vi "Save to File.vi"(8 "error in":errorcluster, 10 "Folder":path, 11 "ILabVIEWFile in":refnum<class "Type Definition.lvclass">) -> (0 "error out":errorcluster, 2 "File Path":path, 3 "ILabVIEWFile out":refnum<class "Type Definition.lvclass">)   [LabVIEW 2026, in "Type Definition.lvclass"]
doc: "Save object to file at the provided path."
uses:
  Type Definition.lvclass
  C:/Users/juanj/Documents/hasbun_wood_engineering/github/py2vi/labview/Classes/LabVIEW File/LabVIEW File.lvclass
  LabVIEW File/LabVIEW File.lvclass/LabVIEW File.ctl
  LabVIEW File/Read VI Reference.vi
  Type Definition.lvclass/Type Definition.ctl
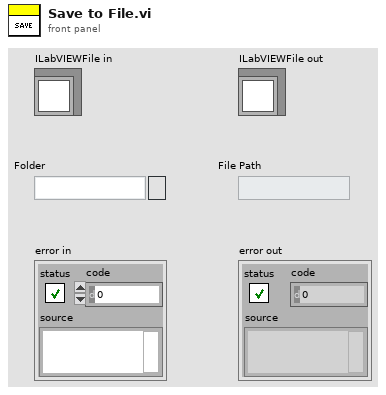
[diagram p1: front panel]
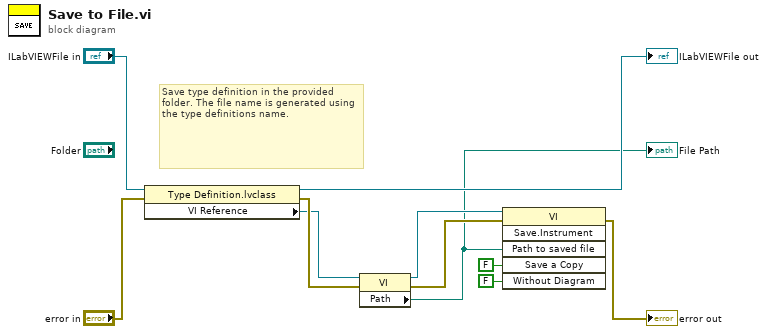
[diagram p0: block diagram]
diagram:
  # "Save type definition in the provided folder. The file name is generated using the type definitions name."
  n1 = property class="Type Definition.lvclass"(reference="ILabVIEWFile in", error in="error in") -> (reference out=→"ILabVIEWFile out":refnum<class "Type Definition.lvclass">, error out=w5:errorcluster, "VI Reference"=w4:refnum<vi>)
  n2 = property class="VI"(reference=w4, error in=w5) -> (reference out=w3:refnum<vi>, error out=w2:errorcluster, "Path"=w1:path)
  "File Path" <- w1
  n3 = invoke on="Invoke Node" class="VI" method="Save.Instrument"(reference=w3, error in=w2, "Path to saved file"=w1, "Save a Copy"=FALSE, "Without Diagram"=FALSE) -> (error out=→"error out":errorcluster)  [unwired: 1 in, 5 out]
